vi "SetTestRbacv3.vi"() -> ()   [LabVIEW 2017]
uses:
  <vilib>/httpClient/PUTBuffer.vi
  <vilib>/httpClient/LabVIEWHTTPClient.lvlib
panel:
  out "data string":string
  out "headers":string
  out "body":string
  out "error out":errorcluster
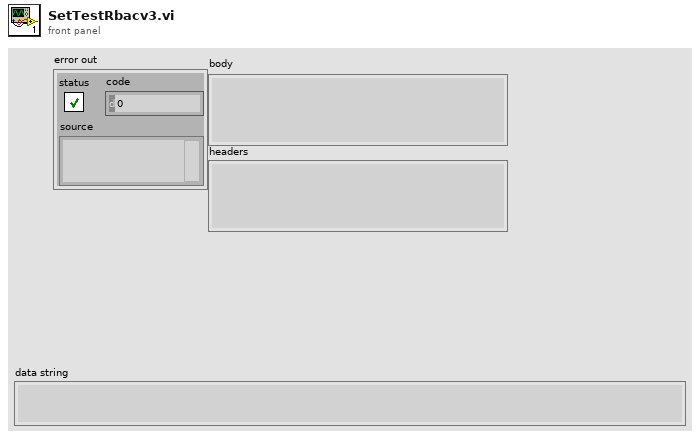
[diagram p1: front panel]
types:
  T1 = typedef "LabVIEWHTTPClient.lvlib/ClientHandle.ctl" = refnum<k1>
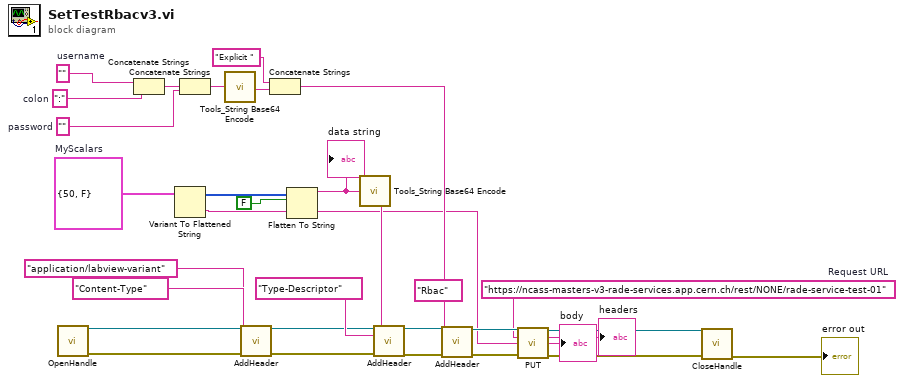
[diagram p0: block diagram]
diagram:
  w4 = "https://ncass-masters-v3-rade-services.app.cern.ch/rest/NONE/rade-service-test-01"  # Request URL
  w26 = ":"  # colon
  w24 = ""  # password
  w27 = ""  # username
  w15 = cluster{"myInt32":i32, "myBoolean":bool} {"myInt32"=50, "myBoolean"=FALSE}  # MyScalars
  n1 = call <vilib>:"OpenHandle.vi"() -> ("client handle out"=w12:T1, "error out"=w11:errorcluster)  [unwired: 14 in]
  n2 = Concatenate Strings(w27, w26) -> (w25:string)
  n3 = Variant To Flattened String(Variant=w15) -> (data string=w3:string, 1:w16:i16[])
  n4 = Concatenate Strings(w25, w24) -> (w22:string)
  n5 = call <userlib>:"Tools_String Base64 Encode.vi"("Normal String"=w22) -> ("Base64 String"=w21:string)  [unwired: 1 in]
  n6 = call <vilib>:"AddHeader.vi"("client handle"=w12, "header"="Content-Type", "value"="application/labview-variant", "error in (no error)"=w11) -> ("client handle out"=w10:T1, "error out"=w9:errorcluster)  [unwired: 10 in]
  n7 = Concatenate Strings("Explicit " ("string"), w21) -> (w20:string)
  n8 = Flatten To String(anything=w16, prepend array or string size? (T)=FALSE) -> (data string=w30:string)  [unwired: 2 in, 2 out]
  "data string" <- w30
  n9 = call <userlib>:"Tools_String Base64 Encode.vi"("Normal String"=w30) -> ("Base64 String"=w29:string)  [unwired: 1 in]
  n10 = call <vilib>:"AddHeader.vi"("client handle"=w10, "header"="Type-Descriptor", "value"=w29, "error in (no error)"=w9) -> ("client handle out"=w19:T1, "error out"=w17:errorcluster)  [unwired: 10 in]
  n11 = call <vilib>:"AddHeader.vi"("client handle"=w19, "header"="Rbac", "value"=w20, "error in (no error)"=w17) -> ("client handle out"=w8:T1, "error out"=w7:errorcluster)  [unwired: 10 in]
  n12 = call-poly <vilib>:"PUT.vi"("client handle"=w8, "url"=w4, "buffer"=w3, "error in (no error)"=w7) -> ("client handle out"=w5:T1, "headers"=→"headers":string, "body"=→"body":string, "error out"=w6:errorcluster)  [unwired: 8 in]
  n13 = call <vilib>:"CloseHandle.vi"("client handle"=w5, "error in (no error)"=w6) -> ("error out"=→"error out":errorcluster)  [unwired: 13 in]
